vi "Check If User Data File is Empty.vi"(8 "error in (no error)":errorcluster, 11 "User Data Path":path) -> (0 "error out":errorcluster)   [LabVIEW 2018]
doc: "Determines whether the user data file is empty or does not contain the expected configuration data. The VI opens the configuration file specified by <b>User Data Path</b> and checks its contents. If the file is empty, it closes the reference, recreates or replaces the file, and initializes it with default user data. The VI propagates any errors through the error cluster."
uses:
  <vilib>/TABOADA/Config Files Management/Config Files Management/config data--cluster.ctl
  <vilib>/Utility/config.llb/NI_LVConfig.lvlib
  <vilib>/TABOADA/Config Files Management/Config Files Management/Config Files Management.lvlib
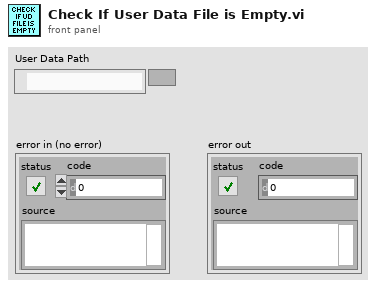
[diagram p1: front panel]
types:
  T1 = typedef "NI_LVConfig.lvlib/Config Data RefNum.ctl" = refnum<k1>
  T2 = typedef "Config Files Management.lvlib/config data--cluster.ctl" = cluster{"sections":string[][], "key names":string[], "values":string[]}
  T3 = enum16{"open", "replace", "create", "open or create", "replace or create", "replace or create with confirmation"}
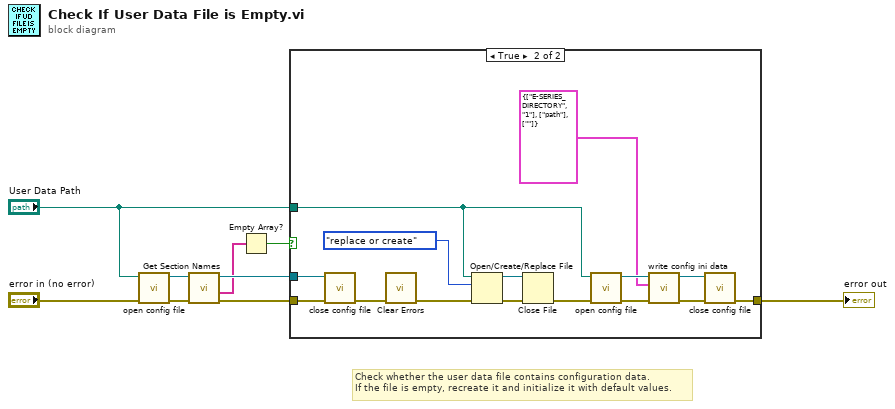
[diagram p0: block diagram]
diagram:
  # "Check whether the user data file contains configuration data.\nIf the file is empty, recreate it and initialize it with default values."
  n1 = call <vilib>:"open config file.vi"("error in (no error)"="error in (no error)", "configuration file path"="User Data Path") -> ("error out"=w3:errorcluster, "Refnum out"=w2:T1)  [unwired: 7 in, 1 out]
  n2 = call <vilib>:"Get Section Names.vi"("error in (no error)"=w3, "refnum"=w2) -> ("error out"=w8:errorcluster, "section names"=w1:string[], "refnum out"=w6:T1)  [unwired: 7 in]
  n3 = Empty Array?(array=w1) -> (empty?=w7:bool)
  n4 = case shown="True" w7 {
    tunnel: w6 -> [_ w11]
    tunnel: w8 -> [w10 w13]
    tunnel: [w10 w16] -> w9
    tunnel: "User Data Path" -> [_ w14]
    frame False {
    }
    frame True {
      n5 = call <vilib>:"close config file.vi"("error in (no error)"=w13, "Refnum in"=w11) -> ("error out"=w12:errorcluster)  [unwired: 9 in]
      n6 = call <vilib>:"Clear Errors.vi"("error in (no error)"=w12) -> ("error out"=w18:errorcluster)  [unwired: 5 in, 1 out]
      n7 = Open/Create/Replace File(file path (use dialog)=w14, error in=w18, operation (0:open)=T3."replace or create") -> (refnum out=w23:refnum<file>, error out=w24:errorcluster)  [unwired: 3 in, 1 out]
      n8 = Close File(refnum=w23, error in=w24) -> (error out=w22:errorcluster)  [unwired: 1 out]
      n9 = call <vilib>:"open config file.vi"("error in (no error)"=w22, "configuration file path"=w14) -> ("error out"=w21:errorcluster, "Refnum out"=w20:T1)  [unwired: 7 in, 1 out]
      n10 = call <vilib>:"write config ini data.vi"("error in (no error)"=w21, "data in"=T2 {"sections"=[["E-SERIES_DIRECTORY"], ["1"]], "key names"=["path"], "values"=[""]} ("User Data"), "Refnum in"=w20) -> ("error out"=w17:errorcluster, "Refnum out"=w15:T1)  [unwired: 7 in]
      n11 = call <vilib>:"close config file.vi"("error in (no error)"=w17, "Refnum in"=w15) -> ("error out"=w16:errorcluster)  [unwired: 9 in]
    }
  }
  "error out" <- w9
